vi "RedistributePathPoints.vi"(0 "IndexedPathLength":dbl[](array[numeric]), 1 "Desired Point Spacing (in)":dbl, 2 "PathIn":T1[](array[typedef]), 3 "Path Length (in)":dbl) -> (5 "IndexedPathLengthOut":dbl[](array[numeric]), 6 "PathOut":T1[](array[typedef]))   [LabVIEW 2018, in "ArgosLib.lvlib"]
uses:
  ArgosLib.lvlib
  TypeDefs/Point2D.ctl
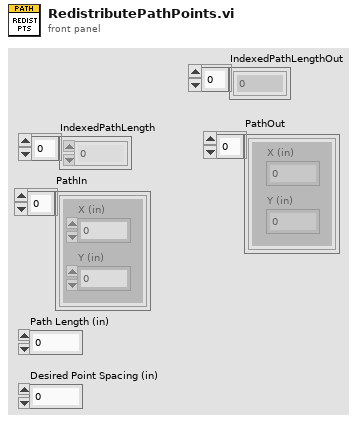
[diagram p1: front panel]
types:
  T1 = typedef "ArgosLib.lvlib/Point2D.ctl" = cluster{"X (in)":dbl, "Y (in)":dbl}
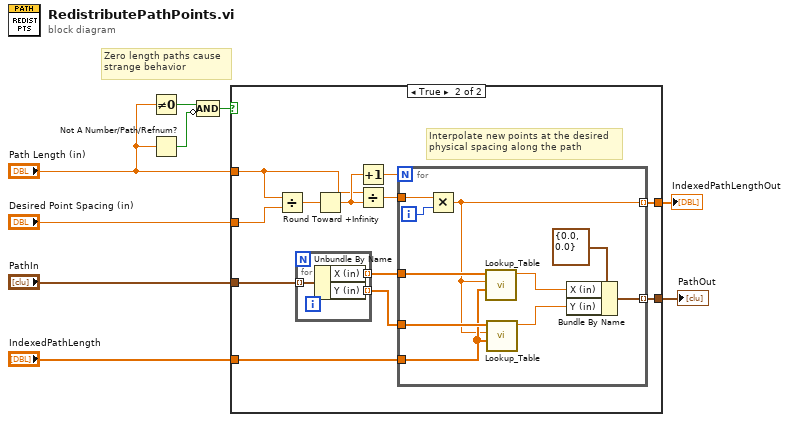
[diagram p0: block diagram]
diagram:
  # "Zero length paths cause\nstrange behavior"
  n1 = Not Equal To 0?(x="Path Length (in)") -> (x != 0?=w5:bool)
  n2 = Not A Number/Path/Refnum?(number/path/refnum="Path Length (in)") -> (NaN/Path/Refnum?=w2:bool)
  n3 = Compound Arithmetic op=AND(w5, invert w2) -> (w4:bool)
  n4 = case shown="True" w4 {
    tunnel: "Desired Point Spacing (in)" -> [_ w23]
    tunnel: "IndexedPathLength" -> [w10 w20]
    tunnel: "PathIn" -> [w11 w18]
    tunnel: [w11 w15] -> w6
    tunnel: "Path Length (in)" -> [_ w13]
    tunnel: [w10 w12] -> w1
    frame False {
      # "Zero length path, just pass through"
    }
    frame True {
      # "Interpolate new points at the desired\nphysical spacing along the path"
      n5 = Divide(x=w13, y=w23) -> (x/y=w22:dbl)
      n6 = for {
        tunnel: w18 -> [w26] mode=indexing
        tunnel: [w25] -> w17 mode=indexing
        tunnel: [w24] -> w16 mode=indexing
        n7 = Unbundle By Name(w26) -> ("X (in)"=w25:dbl, "Y (in)"=w24:dbl)
      }
      n8 = Round Toward +Infinity(x=w22) -> (ceil(x): smallest int >= x=w19:dbl)
      n9 = Increment(x=w19) -> (x+1=w14:dbl)
      n10 = Divide(x=w13, y=w19) -> (x/y=w21:dbl)
      n11 = for {
        N: w14 -> [_]
        tunnel: w21 -> [w35]
        tunnel: w17 -> [w34]
        tunnel: w16 -> [w33]
        tunnel: w20 -> [w32]
        tunnel: [w28] -> w15 mode=indexing
        tunnel: [w27] -> w12 mode=indexing
        i -> [w36]
        n12 = Multiply(x=w35, y=w36) -> (x*y=w27:dbl)
        n13 = call "Lookup_Table.vi"("Y_Array"=w34, "x_in"=w27, "X_Array"=w32) -> ("y_out"=w30:dbl)  [unwired: 6 in]
        n14 = call "Lookup_Table.vi"("Y_Array"=w33, "x_in"=w27, "X_Array"=w32) -> ("y_out"=w29:dbl)  [unwired: 6 in]
        n15 = Bundle By Name(cluster=T1 {"X (in)"=0.0, "Y (in)"=0.0} ("2DPoint"), "X (in)"=w30, "Y (in)"=w29) -> (w28:T1)
      }
    }
  }
  "PathOut" <- w6
  "IndexedPathLengthOut" <- w1
